vi "Actor Core.vi"(8 "error in":errorcluster, 11 "DAQ Timed SPIM in":refnum<class "DAQ Timed SPIM.lvclass">) -> (0 "error out":errorcluster, 3 "Actor out":refnum<class "Actor.lvclass">)   [LabVIEW 2020]
doc: "(<B>Filename</B>: Actor Framework.lvlib:Actor.lvclass:Actor Core.vi)\n\nReceives messages to the actor, reacts to them, and initiates any error handling that may shut the actor down.\n\nDescendant classes may override this VI to append parallel tasks for the actor to complete while it handles messages. Overrides use the Call Parent Class Method node."
uses:
  <vilib>/ActorFramework/Actor/Actor.lvclass
  DAQ Timed SPIM Messages/Stop Triggered Acq Msg/Stop Triggered Acq Msg.lvclass
  DAQ Timed SPIM Messages/Start Triggered Acq Msg/Start Triggered Acq Msg.lvclass
  <vilib>/ActorFramework/Stop Msg/Stop Msg.lvclass
  DAQ Timed SPIM.lvclass
panel:
  in  "Stop Signal":bool
  in  "Stop Button":bool
  in  "Run Button":bool
  in  "Record Button":bool
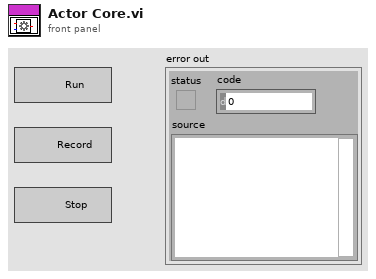
[diagram p1: front panel]
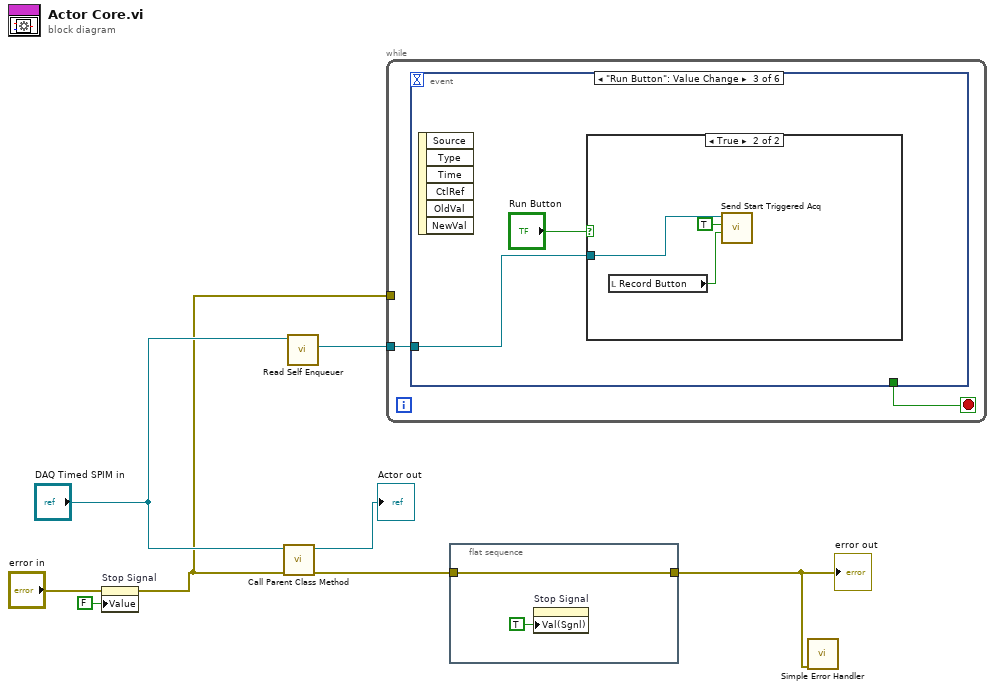
[diagram p0: block diagram]
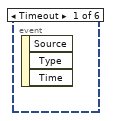
[diagram p2: hidden frame]
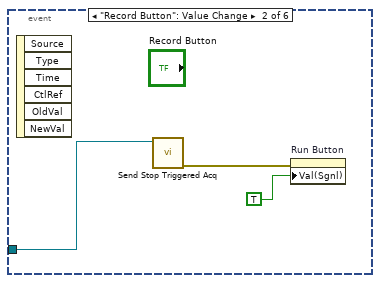
[diagram p3: hidden frame]
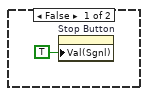
[diagram p4: hidden frame]
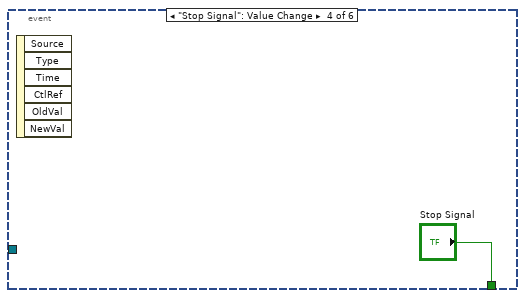
[diagram p5: hidden frame]
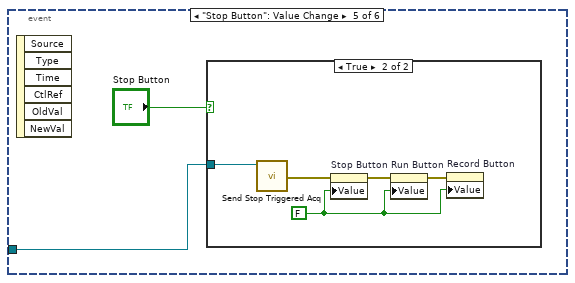
[diagram p6: hidden frame]
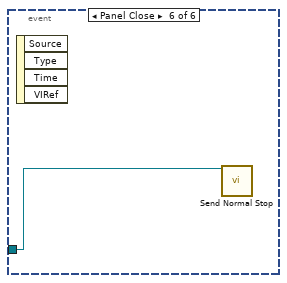
[diagram p8: hidden frame]
diagram:
  n1 = property on="Stop Signal" class="Bool (strict)"(error in="error in", "Value"=FALSE ("Stop Signal")) -> (error out=w2:errorcluster)  [unwired: 1 in, 1 out]
  n2 = call-parent "Call Parent Class Method"("error in"=w2, "Actor in"="DAQ Timed SPIM in") -> ("error out"=w4:errorcluster, "Actor out"=→"Actor out":refnum<class "Actor.lvclass">)  [unwired: 8 in]
  n3 = call <vilib>:"Read Self Enqueuer.vi"("Actor"="DAQ Timed SPIM in") -> ("Self Enqueuer"=w7:refnum<class "Message Enqueuer.lvclass">)  [unwired: 10 in]
  n4 = while {
    tunnel: w7 -> [w10]
    tunnel: w2 -> [_]
    stop <- w9 stop-if-true
    n5 = event shown="[2] \"Run Button\": Value Change" {
      selector: _ -> [_ _ _ _ _ _]
      dyn-events: _ -> [_ _ _ _ _ _]
      timeout: _ -> [_ _ _ _ _ _]
      tunnel: w10 -> [_ w13 w14 _ w22 w28]
      tunnel: [_ _ _ "Stop Signal" _ _] -> w9
      event Timeout {
        n6 = event-data() -> ()  [unwired: 1 in, 3 out]
      }
      event "Record Button": Value Change {
        n7 = event-data() -> ()  [unwired: 1 in, 6 out]
        n8 = call "Send Stop Triggered Acq.vi"("Message Enqueuer"=w13) -> ("error out"=w12:errorcluster)  [unwired: 9 in, 1 out]
        n9 = property on="Run Button" class="Bool (strict)"(error in=w12, "Val(Sgnl)"=TRUE ("Value (Signaling)")) -> ()  [unwired: 1 in, 2 out]
      }
      event "Run Button": Value Change {
        n10 = event-data() -> ()  [unwired: 1 in, 6 out]
        n11 = case shown="True" "Run Button" {
          tunnel: w14 -> [_ w19]
          frame False {
            n12 = property on="Stop Button" class="Bool (strict)"("Val(Sgnl)"=TRUE ("Value (Signaling)")) -> ()  [unwired: 2 in, 2 out]
          }
          frame True {
            n13 = local read "Record Button"() -> (w17:bool)
            n14 = call "Send Start Triggered Acq.vi"("Write to disk?"=w17, "Repeat?"=TRUE, "Message Enqueuer"=w19) -> ()  [unwired: 7 in, 2 out]
          }
        }
      }
      event "Stop Signal": Value Change {
        n15 = event-data() -> ()  [unwired: 1 in, 6 out]
      }
      event "Stop Button": Value Change {
        n16 = event-data() -> ()  [unwired: 1 in, 6 out]
        n17 = case shown="True" "Stop Button" {
          tunnel: w22 -> [_ w27]
          frame False {
          }
          frame True {
            w25 = FALSE ("Stop Button")
            n18 = call "Send Stop Triggered Acq.vi"("Message Enqueuer"=w27) -> ("error out"=w26:errorcluster)  [unwired: 9 in, 1 out]
            n19 = property on="Stop Button" class="Bool (strict)"(error in=w26, "Value"=w25) -> (error out=w24:errorcluster)  [unwired: 1 in, 1 out]
            n20 = property on="Run Button" class="Bool (strict)"(error in=w24, "Value"=w25) -> (error out=w23:errorcluster)  [unwired: 1 in, 1 out]
            n21 = property on="Record Button" class="Bool (strict)"(error in=w23, "Value"=w25) -> ()  [unwired: 1 in, 2 out]
          }
        }
      }
      event Panel Close {
        n22 = event-data() -> ()  [unwired: 1 in, 4 out]
        n23 = call <vilib>:"Send Normal Stop.vi"("Message Enqueuer"=w28) -> ()  [unwired: 10 in, 1 out]
      }
    }
  }
  n24 = flat-sequence {
    tunnel: w4 -> [w29]
    tunnel: [w29] -> w1
    frame #0 {
      n25 = property on="Stop Signal" class="Bool (strict)"("Val(Sgnl)"=TRUE ("Value (Signaling)")) -> ()  [unwired: 2 in, 2 out]
    }
  }
  n26 = call <vilib>:"Simple Error Handler.vi"("error in (no error)"=w1) -> ()  [unwired: 4 in, 5 out]
  "error out" <- w1
